vi "VIH Utility - STR - Remove Duplicated Strings from 1D Array.vi"(8 "error in (no error)":errorcluster, 10 "case sensitive comparison (T)":bool=TRUE, 11 "Array in":string[](array[string])) -> (0 "error out":errorcluster, 3 "Array out":string[](array[string]))   [LabVIEW 2014]
doc: "::: VI Helpeks :::\nCopyright (c) 2000-2026 Konstantin Shifershteyn. All rights reserved."
panel:
  # "VI Helpeks\nCopyright (c) 2012-2026 Konstantin Shifershteyn"
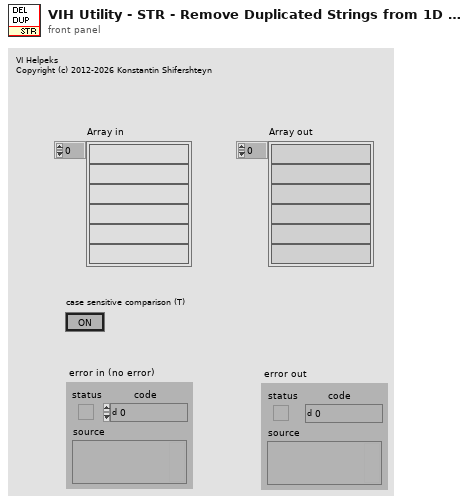
[diagram p1: front panel]
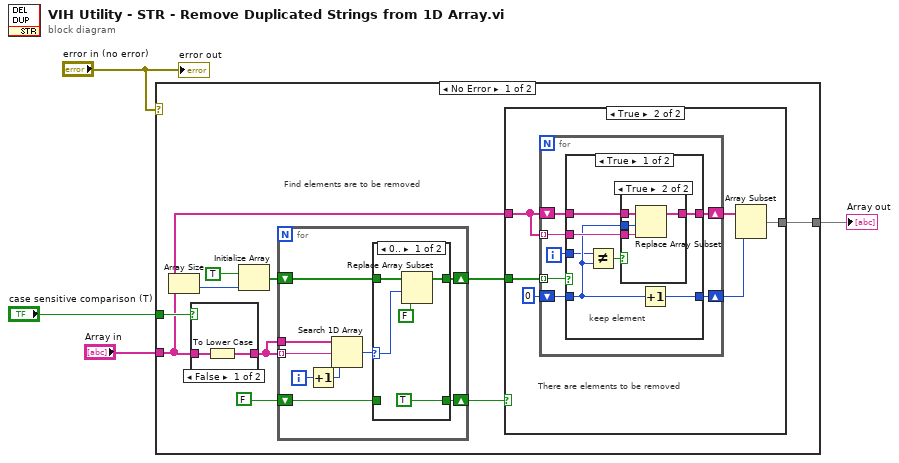
[diagram p0: block diagram]
diagram:
  n1 = case shown="No Error" "error in (no error)" {
    tunnel: "case sensitive comparison (T)" -> [w13 _]
    tunnel: [w10 w62] -> w1
    tunnel: "Array in" -> [w11 w62]
    frame No Error {
      # "Find elements are to be removed"
      n2 = Array Size(array=w11) -> (size(s)=w9:i32)
      n3 = case shown="False" w13 {
        tunnel: [w44 w45] -> w14
        tunnel: w11 -> [w43 w45]
        frame False {
          n4 = To Lower Case(string=w43) -> (all lower case string=w44:string[])
        }
        frame True {
        }
      }
      n5 = Initialize Array(TRUE, w9) -> (w7:bool[])
      n6 = for {
        shift-right: [w49] -> w12
        shift-left: w7 -> [w50]
        tunnel: w14 -> [w54] mode=indexing
        tunnel: w14 -> [w53]
        shift-right: [w46] -> w5
        shift-left: FALSE -> [w47]
        i -> [w48]
        n7 = Increment(x=w48) -> (x+1=w52:i32)
        n8 = Search 1D Array(1D array=w53, element=w54, start index (0)=w52) -> (index of element=w51:i32)
        n9 = case shown="0.." w51 {
          selector: w51 -> [w58 _]
          tunnel: w50 -> [w59 w61]
          tunnel: [w57 w61] -> w49
          tunnel: w47 -> [_ w60]
          tunnel: [TRUE w60] -> w46
          frame 0.. {
            n10 = Replace Array Subset(array=w59, new element=FALSE, index=w58) -> (w57:bool[])
          }
          frame ..-1 {
          }
        }
      }
      n11 = case shown="True" w5 {
        tunnel: w12 -> [_ w18]
        tunnel: w11 -> [w15 w17]
        tunnel: [w15 w16] -> w10
        frame False {
        }
        frame True {
          # "There are elements to be removed"
          n12 = for {
            shift-right: [w26] -> w20
            shift-left: w17 -> [w27]
            tunnel: w18 -> [w28] mode=indexing
            shift-right: [w24] -> w19
            shift-left: 0 -> [w25]
            tunnel: w17 -> [w23] mode=indexing
            i -> [w22]
            n13 = case shown="True" w28 {
              tunnel: w27 -> [w34 w42]
              tunnel: [w33 w42] -> w26
              tunnel: w25 -> [w31 w41]
              tunnel: [w35 w41] -> w24
              tunnel: w23 -> [w32 _]
              tunnel: w22 -> [w30 _]
              frame True {
                # "keep element"
                n14 = Not Equal?(x=w30, y=w31) -> (x != y?=w29:bool)
                n15 = case shown="True" w29 {
                  tunnel: w34 -> [w36 w40]
                  tunnel: [w36 w39] -> w33
                  tunnel: w31 -> [_ w38]
                  tunnel: w32 -> [_ w37]
                  frame False {
                    # "no need\nto\noverwrite"
                  }
                  frame True {
                    n16 = Replace Array Subset(array=w40, new element=w37, index=w38) -> (w39:string[])
                  }
                }
                n17 = Increment(x=w31) -> (x+1=w35:i32)
              }
              frame False {
                # "element is to be removed"
              }
            }
          }
          n18 = Array Subset(array=w20, length=w19) -> (w16:string[])  [unwired: 1 in]
        }
      }
    }
    frame Error {
    }
  }
  "Array out" <- w1
  "error out" <- "error in (no error)"
